vi "Test Context Survives Stuck Owner.vi"(8 "error in (no error)":errorcluster) -> (0 "error out":errorcluster)   [LabVIEW 2019, in "RemoteControl.ZMQ.Tests.lvclass"]
uses:
  RemoteControl.ZMQ.Tests.lvclass
  <vilib>/addons/zeromq/socket_type.ctl
  <vilib>/addons/_JKI Toolkits/Caraya/classes/Test/Test.lvclass
  src/ZMQ.ContextManager/ZMQ.ContextManager.lvlib
  <vilib>/addons/zeromq/zmq_context.lvclass
  <vilib>/addons/zeromq/zeromq.lvlib
  <vilib>/addons/zeromq/zmq_socket.lvclass
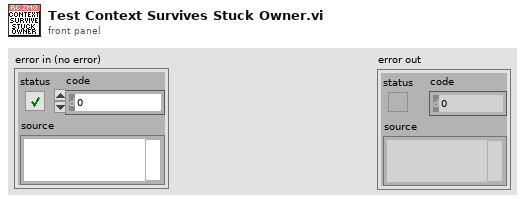
[diagram p1: front panel]
types:
  T1 = typedef "zeromq.lvlib/socket_type.ctl" = enum8{"ZMQ_PAIR", "ZMQ_PUB", "ZMQ_SUB", "ZMQ_REQ", "ZMQ_REP", "ZMQ_DEALER", "ZMQ_ROUTER", "ZMQ_PULL", "ZMQ_PUSH", "ZMQ_XPUB", "ZMQ_XSUB", "ZMQ_STREAM", "ZMQ_SERVER", "ZMQ_CLIENT", "ZMQ_RADIO", "ZMQ_DISH", "ZMQ_GATHER", "ZMQ_SCATTER", "ZMQ_DGRAM"}
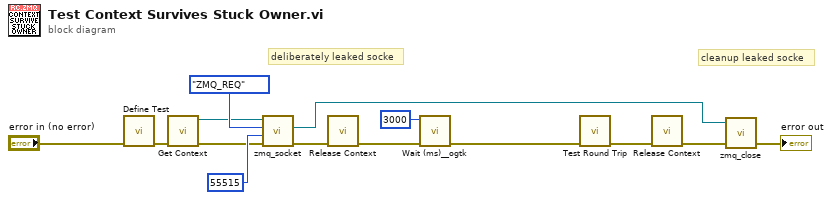
[diagram p0: block diagram]
diagram:
  # "cleanup leaked socke"
  # "deliberately leaked socke"
  n1 = call <vilib>:"Define Test.vi"("error in (no error)"="error in (no error)") -> ("error out"=w2:errorcluster)  [unwired: 9 in, 1 out]
  n2 = call "Get Context.vi"("error in"=w2) -> ("error out"=w11:errorcluster, "context"=w7:refnum<class "zmq_context.lvclass">)  [unwired: 9 in]
  n3 = call <vilib>:"zmq_socket.vi"("error in"=w11, "linger (ms)"=55515, "socket type"=socket_type."ZMQ_REQ", "context in"=w7) -> ("error out"=w10:errorcluster, "socket out"=w4:refnum<class "zmq_socket.lvclass">)  [unwired: 1 in, 1 out]
  n4 = call "Release Context.vi"("error in"=w10) -> ("error out"=w9:errorcluster)  [unwired: 9 in, 1 out]
  n5 = call <userlib>:"Wait (ms)__ogtk.vi"("error in (no error)"=w9, "milliseconds to wait"=u32 3000) -> ("error out"=w1:errorcluster)  [unwired: 8 in, 1 out]
  n6 = call "Test Round Trip.vi"("error in (no error)"=w1) -> ("error out"=w8:errorcluster)  [unwired: 10 in]
  n7 = call "Release Context.vi"("error in"=w8) -> ("error out"=w6:errorcluster)  [unwired: 9 in, 1 out]
  n8 = call <vilib>:"zmq_close.vi"("error in"=w6, "socket"=w4) -> ("error out"=→"error out":errorcluster)  [unwired: 3 in]
